vi "PicoScope5000aGetStreamingValues.vi"(10 "handle in":i16, 11 "error in":errorcluster) -> (0 "Start Index in Driver Buffer":u32, 1 "Trigger":cluster{bool, "triggeredAt (Total samples)":u32}, 2 "handle out":i16, 3 "error out":errorcluster, 4 "Number of Samples":u32, 5 "ready":i16, 6 "Auto Stopped":bool)   [LabVIEW 2016]
doc: "This VI is used in streaming mode to get the latest values from the driver. It should be called in a loop after the oscilloscope has been set up using PicoScope3000aSettings.vi and streaming has been started by calling PicoScope3000aStartStreaming.vi. The VI outputs the number of samples available and the start index of these samples in the array output by PicoScope3000aStartStreaming.vi."
uses:
  ps5000aWrap.dll
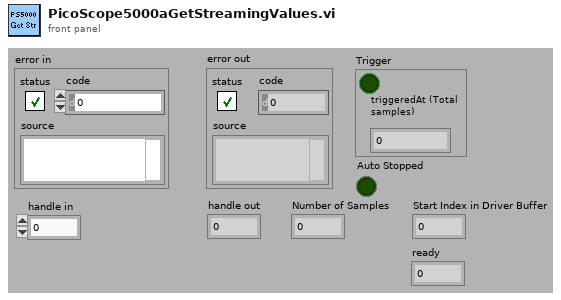
[diagram p1: front panel]
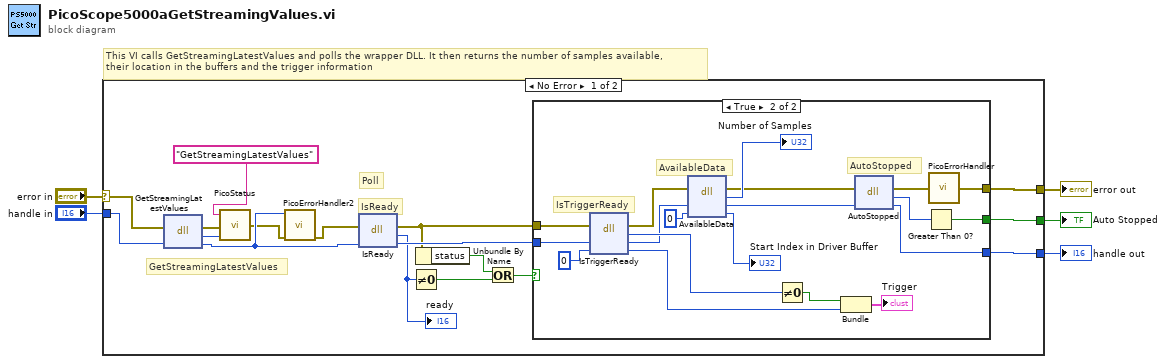
[diagram p0: block diagram]
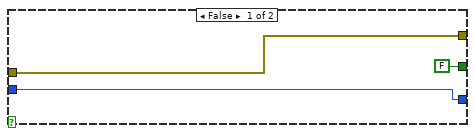
[diagram p2: hidden frame]
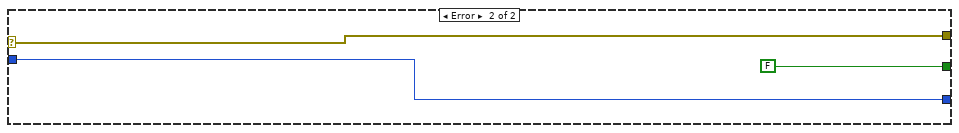
[diagram p3: hidden frame]
diagram:
  # "This VI calls GetStreamingLatestValues and polls the wrapper DLL. It then returns the number of samples available, \ntheir location in the buffers and the trigger information"
  n1 = case shown="No Error" "error in" {
    selector: "error in" -> [w17 w47]
    tunnel: [w22 w47] -> w4
    tunnel: "handle in" -> [w16 w46]
    tunnel: [w19 w46] -> w2
    tunnel: [w18 FALSE] -> w1
    frame No Error {
      # "Poll"
      # "GetStreamingLatestValues"
      # "IsReady"
      n2 = dll-call lib="ps5000aWrap.dll" fn="GetStreamingLatestValues" ("PS5000.dll:_ps5000SetDataBuffer@16")(error in=w17, "handle"=w16) -> (error out=w11:errorcluster, "PICO_STATUS"=w12:u32, "handle"=w9:i16)  [unwired: 2 in, 1 out]
      n3 = call "PicoStatus.vi"("PICO STATUS"=w12, "error in"=w11, "source"="GetStreamingLatestValues") -> ("error out"=w8:errorcluster)
      n4 = call "PicoErrorHandler2.vi"("error in (no error)"=w8, "handle In"=w9) -> ("error out"=w7:errorcluster)  [unwired: 9 in]
      n5 = dll-call lib="ps5000aWrap.dll" fn="IsReady" ("PS5000.dll:_ps5000SetDataBuffer@16")(error in=w7, "handle"=w9) -> (error out=w20:errorcluster, "ready"=w15:i16, "handle"=w21:i16)  [unwired: 2 in, 1 out]
      "ready" <- w15
      n6 = Not Equal To 0?(x=w15) -> (x != 0?=w13:bool)
      n7 = Unbundle By Name(w20) -> ("status"=w14:bool)
      n8 = Or(x=w14, y=w13) -> (x .or. y?=w6:bool)
      n9 = case shown="True" w6 {
        tunnel: [w25 w44] -> w22
        tunnel: w21 -> [w24 w42]
        tunnel: w20 -> [w25 w34]
        tunnel: [w24 w30] -> w19
        tunnel: [FALSE w28] -> w18
        frame False {
        }
        frame True {
          # "AutoStopped"
          # "AvailableData"
          # "IsTriggerReady"
          n10 = dll-call lib="ps5000aWrap.dll" fn="IsTriggerReady" ("PS5000.dll:_ps5000SetDataBuffer@16")(error in=w34, "handle"=w42, "triggeredAt"=u32 0) -> (error out=w38:errorcluster, "triggered"=w41:i16, "handle"=w37:i16, "triggeredAt"=w26:u32)  [unwired: 2 in, 1 out]
          n11 = dll-call lib="ps5000aWrap.dll" fn="AvailableData" ("PS5000.dll:_ps5000Stop@4")(error in=w38, "handle"=w37, "startIndex"=u32 0) -> (error out=w33:errorcluster, "numSamples"=→"Number of Samples":u32, "handle"=w31:i16, "startIndex"=→"Start Index in Driver Buffer":u32)  [unwired: 2 in, 1 out]
          n12 = Not Equal To 0?(x=w41) -> (x != 0?=w40:bool)
          n13 = Bundle(w40, "triggeredAt"=w26) -> (→"Trigger":cluster{bool, "triggeredAt":u32})  [unwired: 1 in]
          n14 = dll-call lib="ps5000aWrap.dll" fn="AutoStopped"(error in=w33, "handle"=w31) -> (error out=w32:errorcluster, "autoStopped"=w29:i16, "handle"=w30:i16)  [unwired: 2 in, 1 out]
          n15 = Greater Than 0?(x=w29) -> (x > 0?=w28:bool)
          n16 = call "PicoErrorHandler.vi"("error in"=w32) -> ("error out"=w44:errorcluster)
        }
      }
    }
    frame Error {
    }
  }
  "error out" <- w4
  "handle out" <- w2
  "Auto Stopped" <- w1
